vi "RepeatFrameBitsToTarget_LP.vi"(8 "target length":dbl, 11 "bit array in":dbl[](array[numeric])) -> (3 "bit array out":dbl[](array[numeric]))   [LabVIEW 2022 SP3]
panel:
  out "ceil(x): smallest int >= x":dbl
  out "x/y":dbl
  out "size(s)":i32
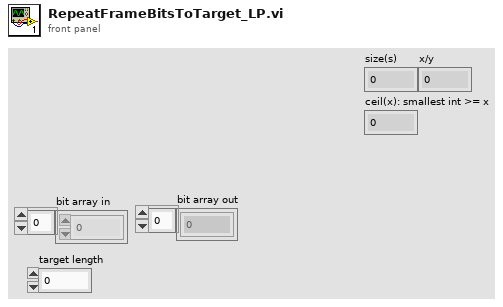
[diagram p1: front panel]
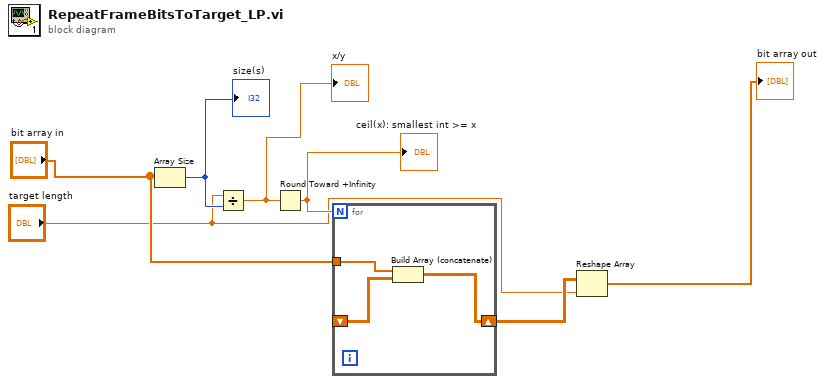
[diagram p0: block diagram]
diagram:
  n1 = Array Size(array="bit array in") -> (size(s)=w7:i32)
  "size(s)" <- w7
  n2 = Divide(x="target length", y=w7) -> (x/y=w6:dbl)
  "x/y" <- w6
  n3 = Round Toward +Infinity(x=w6) -> (ceil(x): smallest int >= x=w5:dbl)
  "ceil(x): smallest int >= x" <- w5
  n4 = for {
    N: w5 -> [_]
    shift-right: [w10] -> w3
    shift-left: _ -> [w8]
    tunnel: "bit array in" -> [w9]
    n5 = Build Array (concatenate)(w9, w8) -> (w10:dbl[][])
  }
  n6 = Reshape Array(w3, "target length") -> (→"bit array out":dbl[])
